vi "Barcode_Scanner_FGV.vi"(3 "error in":errorcluster, 4 "Action":T1, 5 "COM":refnum<visa-resource-name>) -> (0 "error out":errorcluster, 1 "Barcode Data":string, 2 "VISA resource name out":refnum<visa-resource-name>)   [LabVIEW 2021]
uses:
  Control/Barcode.ctl
  <vilib>/Instr/_visa.llb/VISA Configure Serial Port (Instr).vi
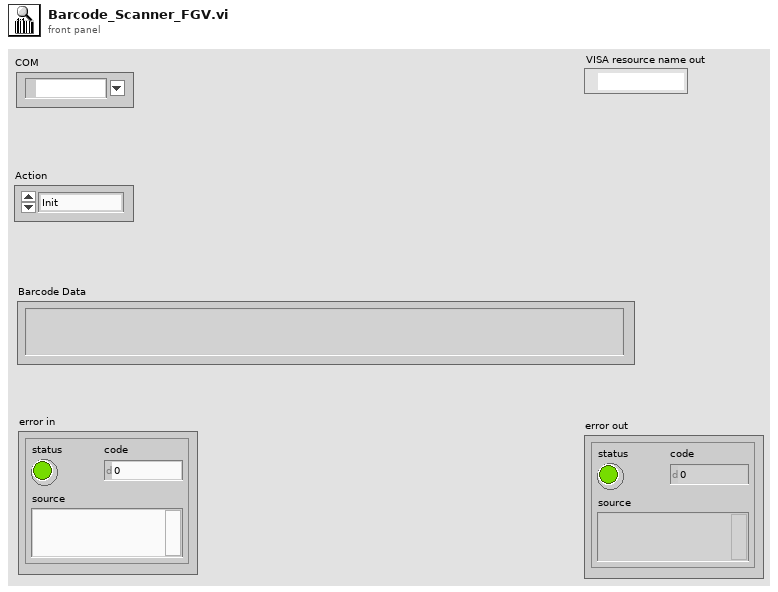
[diagram p1: front panel]
types:
  T1 = typedef "Barcode.ctl" = enum16{"Init", "Read", "Stop Reading", "Clear", "Close"}
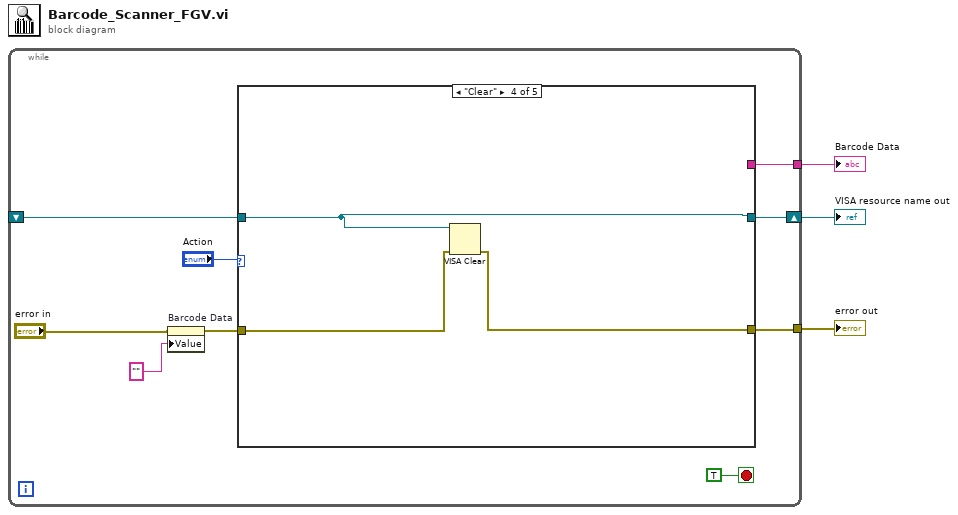
[diagram p0: block diagram]
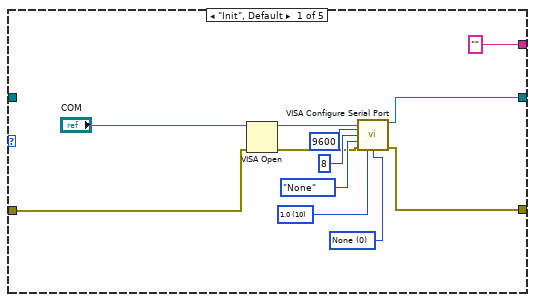
[diagram p2: hidden frame]
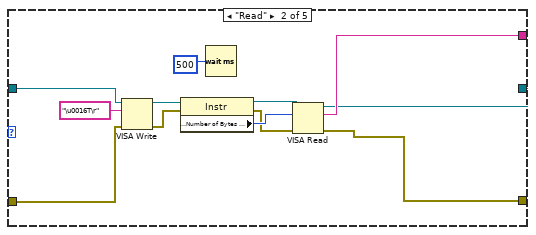
[diagram p3: hidden frame]
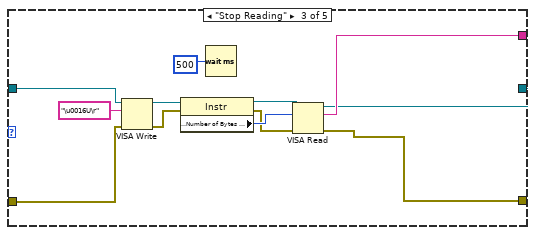
[diagram p4: hidden frame]
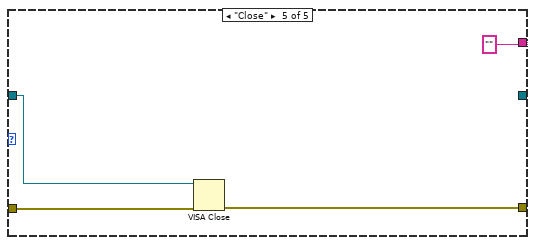
[diagram p5: hidden frame]
diagram:
  n1 = while {
    shift-right: [w11] -> w1
    shift-left: _ -> [w8]
    tunnel: [w10] -> w3
    tunnel: [w9] -> w2
    stop <- TRUE stop-if-true
    n2 = property on="Barcode Data" class="Str"(error in="error in", "Value"="" ("Barcode Data")) -> (error out=w4:errorcluster)  [unwired: 1 in, 1 out]
    n3 = case shown="\"Clear\"" "Action" {
      tunnel: [w18 w26 w38 w51 _] -> w11
      tunnel: w4 -> [w16 w27 w39 w50 w55]
      tunnel: [w15 w25 w37 w49 w53] -> w10
      tunnel: ["" w34 w46 _ ""] -> w9
      tunnel: w8 -> [_ w28 w40 w51 w52]
      frame "Init", Default {
        w19 = u16 0 items=["None", "XON/XOFF", "RTS/CTS", "XON/XOFF & RTS/CTS", "DTR/DSR", "XON/XOFF & DTR/DSR"] ("flow control (0:none)")
        w20 = u16 10 items=["1.0"=10, "1.5"=15, "2.0"=20] ("stop bits (10: 1 bit)")
        n4 = VISA Open(error in (no error)=w16, VISA resource name="COM") -> (VISA resource name=w24:refnum<visa-resource-name>, error out=w17:errorcluster)  [unwired: 3 in]
        n5 = call-poly "VISA Configure Serial Port"("VISA resource name"=w24, "baud rate (9600)"=u32 9600, "data bits (8)"=u16 8, "parity (0:none)"=enum16{"None", "Odd", "Even", "Mark", "Space"}."None", "error in (no error)"=w17, "stop bits (10: 1 bit)"=w20, "flow control (0:none)"=w19) -> ("VISA resource name out"=w18:refnum<visa-resource-name>, "error out"=w15:errorcluster)  [unwired: 7 in]
      }
      frame "Read" {
        n6 = VISA Write(VISA resource name=w28, write buffer="\u0016T\r", error in (no error)=w27) -> (VISA resource name out=w29:refnum<visa-resource-name>, error out=w30:errorcluster)  [unwired: 1 out]
        n7 = property class="Instr"(reference=w29, error in=w30) -> (reference out=w35:refnum<visa-resource-name>, error out=w33:errorcluster, "Serial Settings:Number of Bytes at Serial Port"=w36:u32)
        n8 = Wait (ms)(milliseconds to wait=u32 500) -> ()  [unwired: 1 out]
        n9 = VISA Read(VISA resource name=w35, byte count=w36, error in (no error)=w33) -> (VISA resource name out=w26:refnum<visa-resource-name>, read buffer=w34:string, error out=w25:errorcluster)  [unwired: 1 out]
      }
      frame "Stop Reading" {
        n10 = VISA Write(VISA resource name=w40, write buffer="\u0016U\r", error in (no error)=w39) -> (VISA resource name out=w41:refnum<visa-resource-name>, error out=w42:errorcluster)  [unwired: 1 out]
        n11 = property class="Instr"(reference=w41, error in=w42) -> (reference out=w47:refnum<visa-resource-name>, error out=w45:errorcluster, "Serial Settings:Number of Bytes at Serial Port"=w48:u32)
        n12 = Wait (ms)(milliseconds to wait=u32 500) -> ()  [unwired: 1 out]
        n13 = VISA Read(VISA resource name=w47, byte count=w48, error in (no error)=w45) -> (VISA resource name out=w38:refnum<visa-resource-name>, read buffer=w46:string, error out=w37:errorcluster)  [unwired: 1 out]
      }
      frame "Clear" {
        n14 = VISA Clear(VISA resource name=w51, error in (no error)=w50) -> (error out=w49:errorcluster)  [unwired: 1 out]
      }
      frame "Close" {
        n15 = VISA Close(VISA resource name=w52, error in (no error)=w55) -> (error out=w53:errorcluster)
      }
    }
  }
  "Barcode Data" <- w2
  "error out" <- w3
  "VISA resource name out" <- w1
